vi "Start Acquisition.vi"(8 "error in (no error)":errorcluster, 11 "ImageHandler:DT-ImageHandler in":refnum<class "DT-ImageHandler.lvclass">) -> (0 "error out":errorcluster, 2 "function return":i32, 3 "ImageHandler:DT-ImageHandler out":refnum<class "DT-ImageHandler.lvclass">)   [LabVIEW 2022 SP3, in "ImageHandler.lvlib" / "DT-ImageHandler.lvclass"]
uses:
  DT-ImageHandler.lvclass
  DT-ImageHandler.lvclass/DT-ImageHandler.ctl
  xPanelWrapperLvLib/xPanelWrapper.lvlib
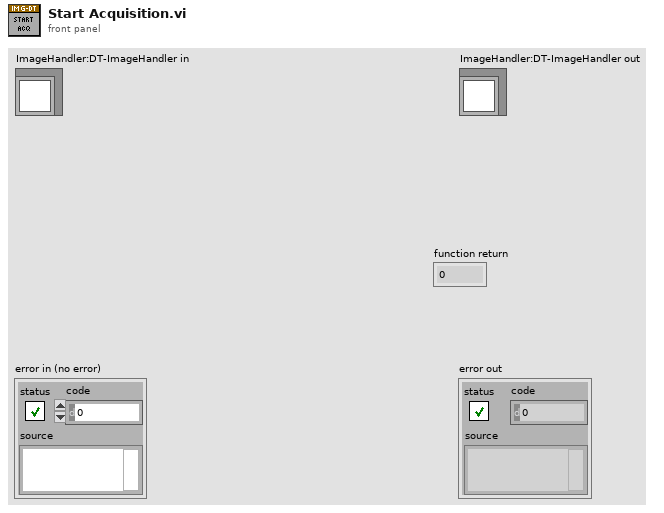
[diagram p1: front panel]
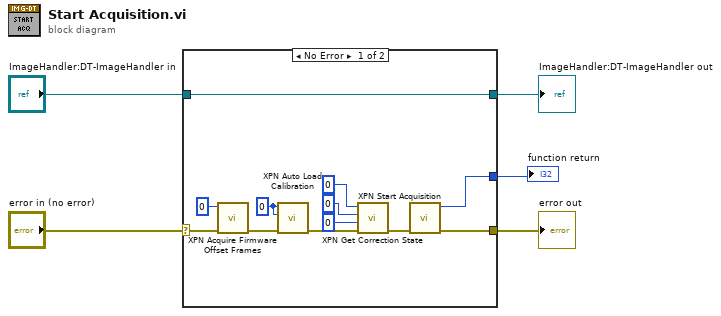
[diagram p0: block diagram]
diagram:
  n1 = case shown="No Error" "error in (no error)" {
    selector: "error in (no error)" -> [w17 w18]
    tunnel: [w16 w18] -> w4
    tunnel: [w15 w19] -> w3
    tunnel: "ImageHandler:DT-ImageHandler in" -> [w15 w19]
    tunnel: [w6 _] -> w1
    frame No Error {
      w10 = 0 ("offsetLoaded")
      n2 = call "XPN Acquire Firmware Offset Frames.vi"("error in (no error)"=w17, "numFrames"=0) -> ("error out"=w12:errorcluster)  [unwired: 8 in, 1 out]
      n3 = call "XPN Auto Load Calibration.vi"("error in (no error)"=w12, "gainLoaded"=w10, "offsetLoaded"=w10) -> ("error out"=w14:errorcluster)  [unwired: 5 in, 3 out]
      n4 = call "XPN Get Correction State.vi"("error in (no error)"=w14, "defectMode"=0 ("offsetLoaded"), "gainMode"=0 ("offsetLoaded"), "offsetMode"=0 ("offsetLoaded")) -> ("error out"=w13:errorcluster)  [unwired: 3 in, 4 out]
      n5 = call "XPN Start Acquisition.vi"("error in (no error)"=w13) -> ("error out"=w16:errorcluster, "function return"=w6:i32)  [unwired: 9 in]
    }
    frame Error {
    }
  }
  "error out" <- w4
  "ImageHandler:DT-ImageHandler out" <- w3
  "function return" <- w1
